vi "isConnected.vi"(8 "error in (no error)":errorcluster, 11 "Client in":refnum<class "Client.lvclass">) -> (0 "error out":errorcluster, 2 "connected":bool, 3 "Client out":refnum<class "Client.lvclass">)   [LabVIEW 2013, in "MQTT Client.lvlib" / "Client.lvclass"]
uses:
  Client.lvclass
  Client.lvclass/Client.ctl
  <vilib>/LabVIEW Open Source Project/MQTT Connection/MQTT_Base/Session/Session.lvclass
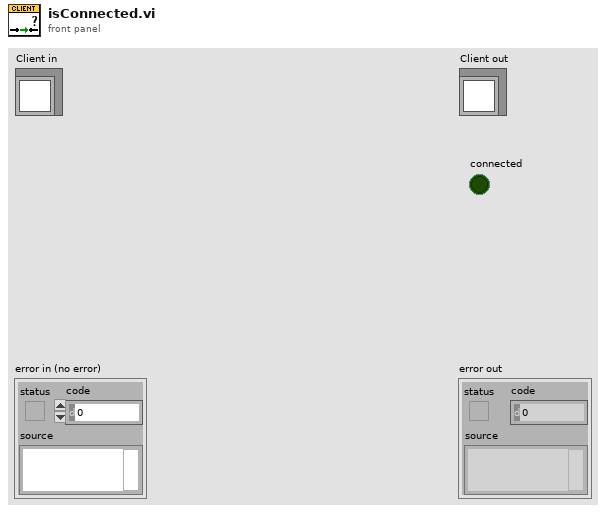
[diagram p1: front panel]
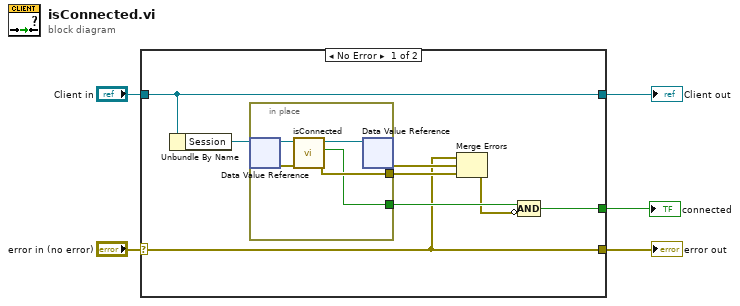
[diagram p0: block diagram]
diagram:
  n1 = case shown="No Error" "error in (no error)" {
    selector: "error in (no error)" -> [w7 w20]
    tunnel: [w7 w20] -> w4
    tunnel: [w9 w19] -> w2
    tunnel: "Client in" -> [w9 w19]
    tunnel: [w13 _] -> w1
    frame No Error {
      n2 = Unbundle By Name(w9) -> ("Session"=w12:refnum<data-value>)
      n3 = in-place {
        in-place-border: [w15] -> w10
        in-place-border: [w14] -> w8
        n4 = in-place-dvr #1(w12) -> (w18:refnum<class "Session.Client.lvclass">, w16:errorcluster)
        n5 = call <vilib>:"isConnected.vi"("error in (no error)"=w16, "Session in"=w18) -> ("error out"=w15:errorcluster, "connected"=w14:bool, "Session out"=w17:refnum<class "Session.Client.lvclass">)  [unwired: 7 in]
        n6 = in-place-dvr #1(w17) -> (w11:errorcluster)  [unwired: 1 out]
      }
      n7 = Merge Errors(w7, w11, w10) -> (w6:errorcluster)
      n8 = Compound Arithmetic op=AND(w8, invert w6) -> (w13:bool)
    }
    frame Error {
    }
  }
  "error out" <- w4
  "Client out" <- w2
  "connected" <- w1
